vi "Get U64 Package Attribute Value.vi"(8 "error in (no error)":errorcluster, 10 "package attribute name":string, 11 "package attributes CLI string":string) -> (0 "error out":errorcluster, 1 "attribute found?":bool, 3 "package attribute value":u64)   [LabVIEW 2014, in "NIPM_API.lvlib"]
doc: "Gets the value for a U64 attribute in a package attribute string.\n\nINPUT(s)\n<B>Package attributes string in</B>: This is the initial string containing the package attributes and values. For example, this string could come from the output of a nipkg CLI command.\n\n<B>Package attribute name</B>: This is the name of the attribute whose value you want to change.\n\nOUTPUT(s)\n<B>Package attribute value</B>: This is the value of the specified attribute.\n\n<B>Attribute found?</B>: Returns whether the attribute was found"
uses:
  NIPM_API.lvlib
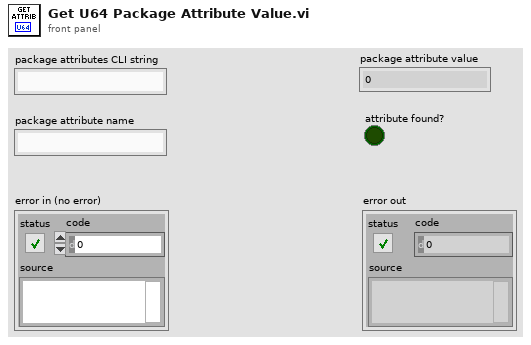
[diagram p1: front panel]
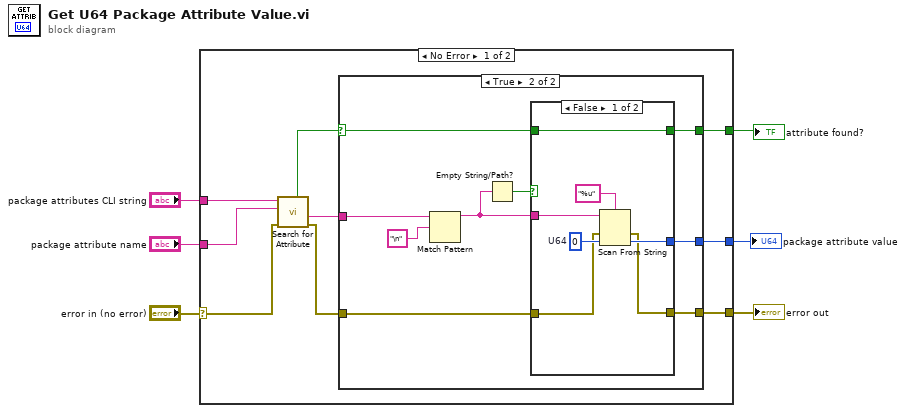
[diagram p0: block diagram]
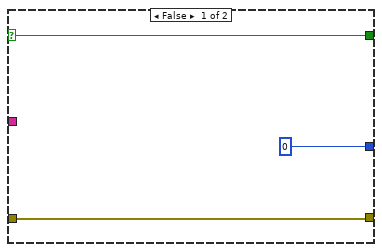
[diagram p2: hidden frame]
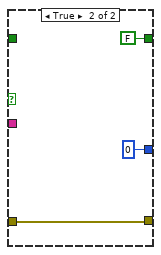
[diagram p3: hidden frame]
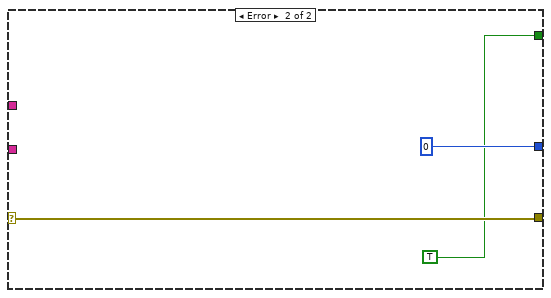
[diagram p4: hidden frame]
diagram:
  n1 = case shown="No Error" "error in (no error)" {
    selector: "error in (no error)" -> [w11 w39]
    tunnel: "package attribute name" -> [w12 _]
    tunnel: "package attributes CLI string" -> [w13 _]
    tunnel: [w15 u64 0 ("U64")] -> w4
    tunnel: [w14 w39] -> w2
    tunnel: [w9 TRUE ("attribute found?")] -> w1
    frame No Error {
      n2 = call "Search for Attribute.vi"("error in (no error)"=w11, "package attribute name"=w12, "package attributes CLI string in"=w13) -> ("error out"=w10:errorcluster, "string after attribute"=w7:string, "attribute found?"=w8:bool)  [unwired: 3 in, 3 out]
      n3 = case shown="True" w8 {
        selector: w8 -> [w16 w19]
        tunnel: [u64 0 ("U64") w26] -> w15
        tunnel: [w18 w24] -> w14
        tunnel: w7 -> [_ w22]
        tunnel: w10 -> [w18 w21]
        tunnel: [w16 w20] -> w9
        frame False {
        }
        frame True {
          n4 = Match Pattern(string=w22, regular expression="\n") -> (before substring=w25:string)  [unwired: 1 in, 3 out]
          n5 = Empty String/Path?(string/path=w25) -> (empty?=w23:bool)
          n6 = case shown="False" w23 {
            tunnel: [w32 u64 0 ("U64")] -> w26
            tunnel: w25 -> [w31 _]
            tunnel: w21 -> [w30 w36]
            tunnel: [w29 w36] -> w24
            tunnel: [w28 FALSE ("attribute found?")] -> w20
            tunnel: w19 -> [w28 _]
            frame False {
              w33 = u64 0  # U64
              n7 = Scan From String(format string="%u", input string=w31, error in=w30, default 1=w33) -> (error out=w29:errorcluster, output 1=w32:u64)  [unwired: 1 in, 2 out]
            }
            frame True {
            }
          }
        }
      }
    }
    frame Error {
    }
  }
  "package attribute value" <- w4
  "error out" <- w2
  "attribute found?" <- w1
